vi "Max_rr_base change.vi"(10 "Numeric":i32=5, 11 "S New Info and MiN":T1={"Sample Sequence"="GATGATGATGATGATGAT", "Right Read MIN"=6, "Filter P"=0, "STD Type"=enum."Region", "Base Table"=[], "Selection"=enum."10kHz", "noise MAX"=3, "Sample name"="(GAT)x6"} {"Base Table"."Value 3" format="%.2g"}) -> (3 "S New Info and MiN 2":T1={"Sample Sequence"="GATGATGATGATGATGAT", "Right Read MIN"=6, "Filter P"=0, "STD Type"=enum."Region", "Base Table"=[], "Selection"=enum."10kHz", "noise MAX"=3, "Sample name"="(GAT)x6"} {"Base Table"."Value 3" format="%.2g"})   [LabVIEW 2018]
panel:
  out "Sample Sequence":string
  out "Selection":enum16{"10kHz", "100kHz"}(ring)
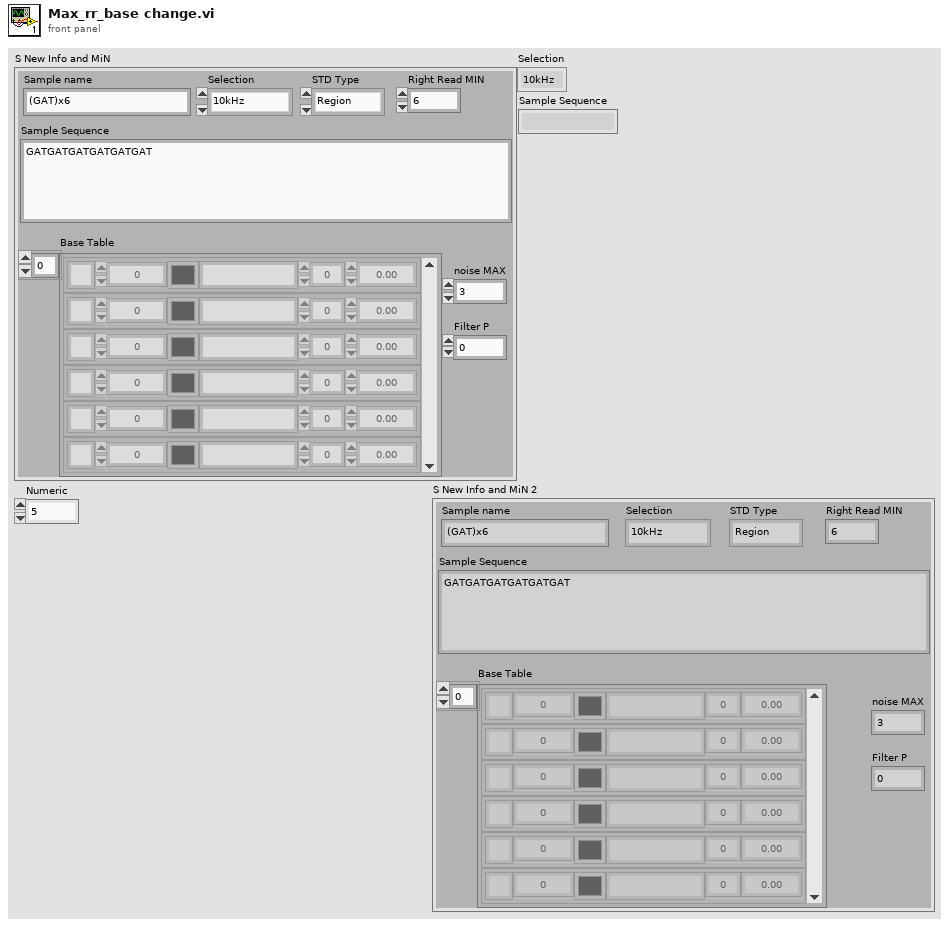
[diagram p1: front panel]
types:
  T1 = cluster{"Sample Sequence":string, "Right Read MIN":i32, "Filter P":i32, "STD Type":enum16{"Region", "Each", "Fixed"}, "Base Table":cluster{"Name":string, "Value":dbl, "Color":u32, "Name 2":string, "Value 2":dbl, "Value 3":dbl}[], "Selection":enum16{"10kHz", "100kHz"}, "noise MAX":i32, "Sample name":string}
  T2 = cluster{"Name":string, "Value":dbl, "Color":u32, "Name 2":string, "Value 2":dbl, "Value 3":dbl}[]
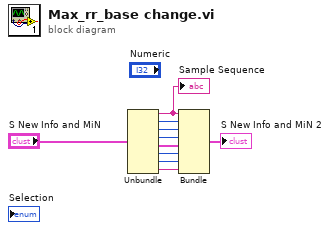
[diagram p0: block diagram]
diagram:
  n1 = Unbundle("S New Info and MiN") -> ("Sample Sequence"=w8:string, "Right Read MIN"=w1:i32, "Filter P"=w2:i32, "STD Type"=w7:enum16{"Region", "Each", "Fixed"}, "Base Table"=w6:T2, "Selection"=w5:enum16{"10kHz", "100kHz"}, "noise MAX"=w4:i32, "Sample name"=w3:string)
  "Sample Sequence" <- w8
  n2 = Bundle("Sample Sequence"=w8, "Right Read MIN"=w1, "Filter P"=w2, "STD Type"=w7, "Base Table"=w6, "Selection"=w5, "noise MAX"=w4, "Sample name"=w3) -> (→"S New Info and MiN 2":T1)  [unwired: 1 in]
